vi "RDC-Array-Reflection_Correction.vi"(7 "e gamma mix":cdb[](array[numeric]), 11 "Measured":T1) -> (2 "Reflection":cdb[](array[numeric]), 3 "Tip":T1)   [LabVIEW 2020, in "RDC-Reflection_Data_Computation.lvlib"]
doc: "Applies the e gamma mix array to the measured reflection of a Common Format cluster. Returns the corrected reflection array and the Tip Common Format cluster with Reflection' and Reflection'' replaced."
uses:
  RDC-Reflection_Data_Computation.lvlib
  Reflector/RFH-common_data_format.ctl
  Reflector/RFH-Reflection_File_Handler.lvlib
panel:
  out "Reflection 2":dbl[][](graph)
  out "Reflection":dbl[][](graph)
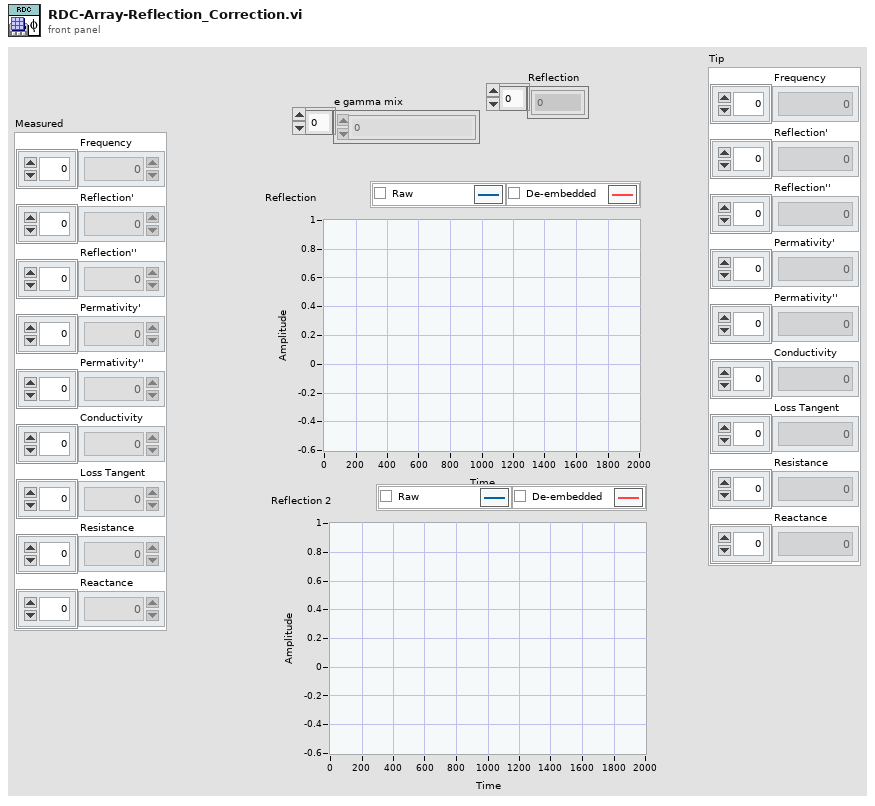
[diagram p1: front panel]
types:
  T1 = typedef "RFH-Reflection_File_Handler.lvlib/RFH-common_data_format.ctl" = cluster{"Frequency":dbl[], "Reflection'":dbl[], "Reflection''":dbl[], "Permativity'":dbl[], "Permativity''":dbl[], "Conductivity":dbl[], "Loss Tangent":dbl[], "Resistance":dbl[], "Reactance":dbl[]}
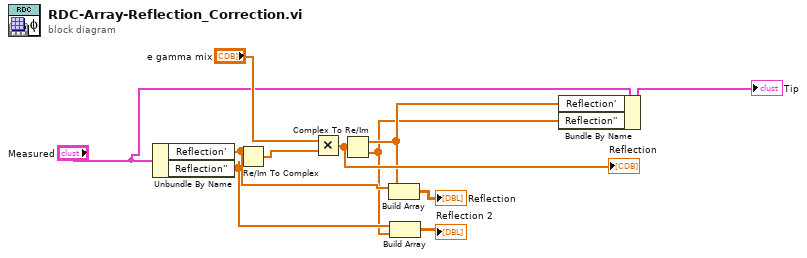
[diagram p0: block diagram]
diagram:
  n1 = Unbundle By Name("Measured") -> ("Reflection'"=w8:dbl[], "Reflection''"=w7:dbl[])
  n2 = Re/Im To Complex(1:w7, 2:w8) -> (0:w11:cdb[])
  n3 = Multiply(x="e gamma mix", y=w11) -> (x*y=w9:cdb[])
  "Reflection" <- w9
  n4 = Complex To Re/Im(x + iy=w9) -> (x=w2:dbl[], y=w1:dbl[])
  n5 = Build Array(w8, w2) -> (→"Reflection":dbl[][])
  n6 = Build Array(w7, w1) -> (→"Reflection 2":dbl[][])
  n7 = Bundle By Name(cluster="Measured", "Reflection'"=w2, "Reflection''"=w1) -> (→"Tip":T1)
